vi "Write Spectrum Device Type.vi"(8 "error in (no error)":errorcluster, 10 "Spectrum Device Type":T1, 11 "FSV-40N in":refnum<class "FSV-40N.lvclass">) -> (0 "error out":errorcluster, 3 "FSV-40N out":refnum<class "FSV-40N.lvclass">)   [LabVIEW 2023, in "Spectrum Analyzer.lvlib" / "FSV-40N.lvclass"]
uses:
  FSV-40N.lvclass
  FSV-40N.lvclass/FSV-40N.ctl
  TYPE DEFINITION/TYPE Supported Spectrum Device Type.ctl
  Spectrum Analyzer.lvlib
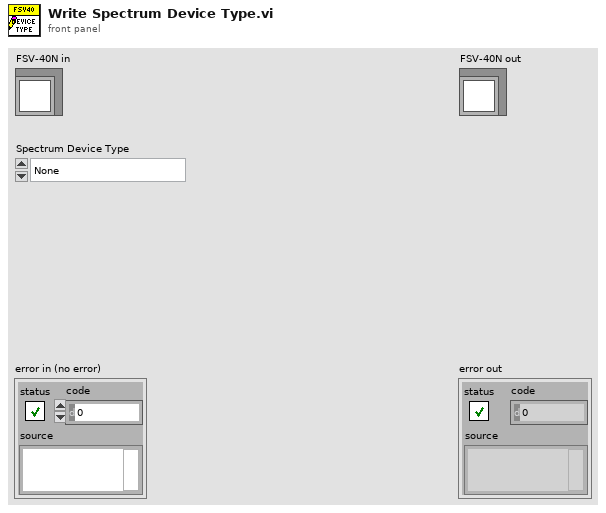
[diagram p1: front panel]
types:
  T1 = typedef "Spectrum Analyzer.lvlib/TYPE Supported Spectrum Device Type.ctl" = enum16{"None", "FSV-30", "FSV-40", "FSW", "9020A"}
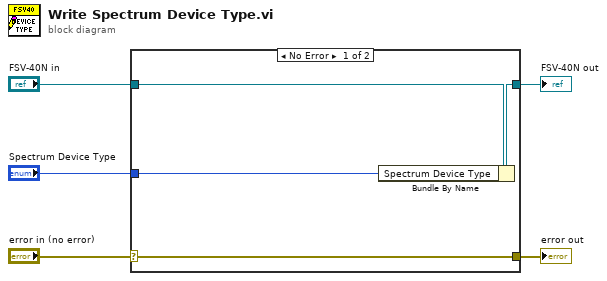
[diagram p0: block diagram]
diagram:
  n1 = case shown="No Error" "error in (no error)" {
    selector: "error in (no error)" -> [w9 w10]
    tunnel: [w9 w10] -> w4
    tunnel: [w7 w11] -> w2
    tunnel: "FSV-40N in" -> [w8 w11]
    tunnel: "Spectrum Device Type" -> [w6 _]
    frame No Error {
      n2 = Bundle By Name(cluster=w8, "Spectrum Device Type"=w6) -> (w7:refnum<class "FSV-40N.lvclass">)
    }
    frame Error {
    }
  }
  "error out" <- w4
  "FSV-40N out" <- w2
